vi "RT DAQ Settings.vi"(8 "error in (no error)":errorcluster, 9 "DAQ Trigger":T1={"Trig Source"=0, "Digital Trigger"=FALSE, "Trig Edge"=10171, "Pulse Line"=0, "Pulse On Time"=0} {"Pulse Line" items=["/Line0", "/Line1", "/Line2", "/Line3", "/Line4", "/Line5", "/Line6", "/Line7", "/Line8", "/Line9", "/Line10", "/Line11", "/Line12", "/Line13", "/Line14", "/Line15"]; "Trig Edge" items=["Rising"=10280, "Falling"=10171]; "Trig Source" items=["PFI0", "PFI1", "PFI2", "PFI3", "PFI4", "PFI5", "PFI6", "PFI7", "PFI8", "PFI9", "PFI10", "PFI11", "PFI12", "PFI13", "PFI14", "PFI15"]}, 10 "DAQ Timing":T2={"Number of Samples"=40000, "Samples Per Second"=970000.0, "Sample Mode"=10178, "Timeout (s)"=10.0} {"Sample Mode" items=["Continuous"=10123, "Finite Sample"=10178, "Hardware Timed Single Point"=12522]}, 11 "DAQ Channel":T3={"Channel"=1, "input terminal configuration"=10106, "Input Range Range"=10.0, "Device"="DAQ1"} {"input terminal configuration" items=["default"=-1, "RSE"=10083, "NRSE"=10078, "Differential"=10106, "Pseudodifferential"=12529]; "Input Range Range" items=["+/-10V"=10.0, "+/-5V"=5.0, "+/-2V"=2.0, "+/-1V"=1.0, "+/-0.5V"=0.5, "+/-0.2V"=0.2, "+/-0.1V"=0.1]; "Channel" items=["0"=0, "1"=1, "2"=2, "3"=3, "4"=4, "5"=5, "6"=6, "7"=7, "16"=16, "17"=17, "18"=18, "19"=19, "20"=20, "21"=21, "22"=22, "23"=23]}) -> (0 "error out":errorcluster, 1 "DAQ Trigger Out":T1={"Trig Source"=0, "Digital Trigger"=FALSE, "Trig Edge"=10171, "Pulse Line"=0, "Pulse On Time"=0} {"Pulse Line" items=["/Line0", "/Line1", "/Line2", "/Line3", "/Line4", "/Line5", "/Line6", "/Line7", "/Line8", "/Line9", "/Line10", "/Line11", "/Line12", "/Line13", "/Line14", "/Line15"]; "Trig Edge" items=["Rising"=10280, "Falling"=10171]; "Trig Source" items=["PFI0", "PFI1", "PFI2", "PFI3", "PFI4", "PFI5", "PFI6", "PFI7", "PFI8", "PFI9", "PFI10", "PFI11", "PFI12", "PFI13", "PFI14", "PFI15"]}, 2 "DAQ Timing Out":T2={"Number of Samples"=40000, "Samples Per Second"=970000.0, "Sample Mode"=10178, "Timeout (s)"=10.0} {"Sample Mode" items=["Continuous"=10123, "Finite Sample"=10178, "Hardware Timed Single Point"=12522]}, 3 "DAQ Channel  Out":T3={"Channel"=1, "input terminal configuration"=10106, "Input Range Range"=10.0, "Device"="DAQ1"} {"input terminal configuration" items=["default"=-1, "RSE"=10083, "NRSE"=10078, "Differential"=10106, "Pseudodifferential"=12529]; "Input Range Range" items=["+/-10V"=10.0, "+/-5V"=5.0, "+/-2V"=2.0, "+/-1V"=1.0, "+/-0.5V"=0.5, "+/-0.2V"=0.2, "+/-0.1V"=0.1]; "Channel" items=["0"=0, "1"=1, "2"=2, "3"=3, "4"=4, "5"=5, "6"=6, "7"=7, "16"=16, "17"=17, "18"=18, "19"=19, "20"=20, "21"=21, "22"=22, "23"=23]}, 7 "DAQ Pusle Out":T4)   [LabVIEW 2013]
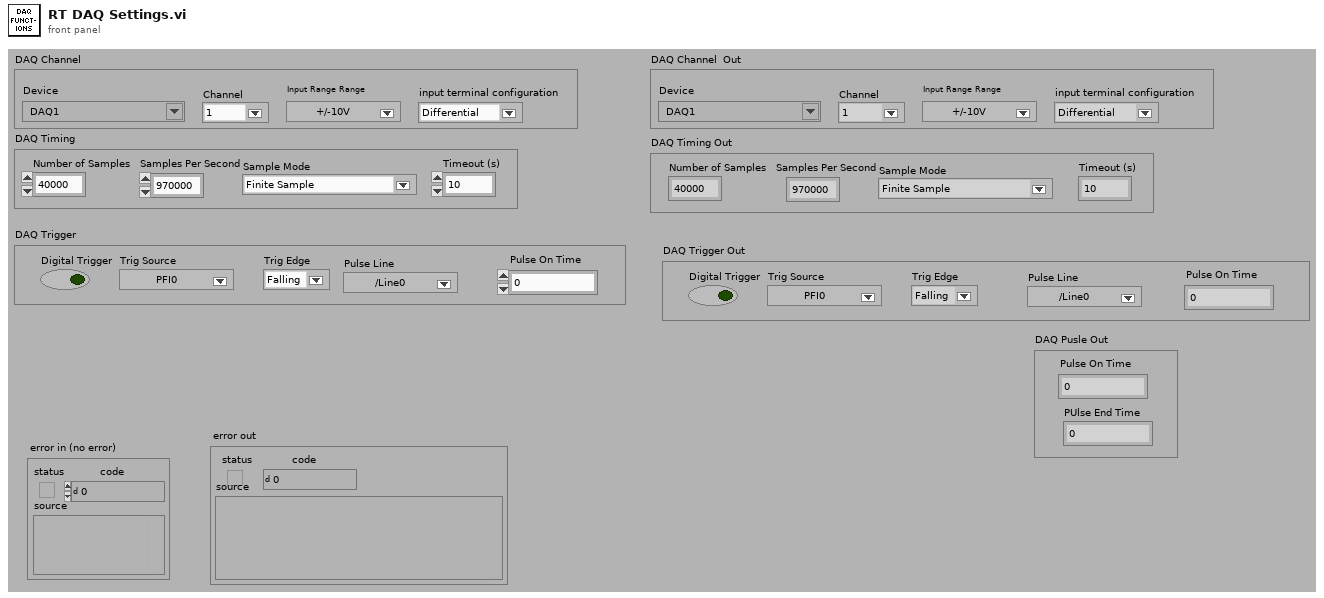
[diagram p1: front panel]
types:
  T1 = cluster{"Trig Source":u16, "Digital Trigger":bool, "Trig Edge":i32, "Pulse Line":u16, "Pulse On Time":u32}
  T2 = cluster{"Number of Samples":u32, "Samples Per Second":dbl, "Sample Mode":i32, "Timeout (s)":dbl}
  T3 = cluster{"Channel":u16, "input terminal configuration":i32, "Input Range Range":dbl, "Device":string}
  T4 = cluster{"Pulse On Time":u32, "PUlse End Time":u32}
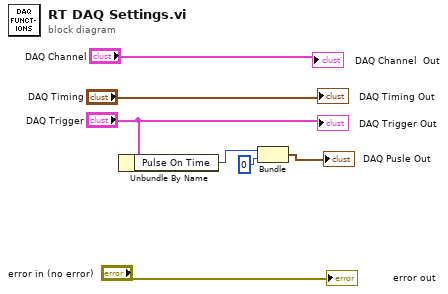
[diagram p0: block diagram]
diagram:
  n1 = Unbundle By Name("DAQ Trigger") -> ("Pulse On Time"=w2:u32)
  n2 = Bundle("Pulse On Time"=w2, 0) -> (→"DAQ Pusle Out":cluster{"Pulse On Time":u32, i32})  [unwired: 1 in]
  "error out" <- "error in (no error)"
  "DAQ Channel  Out" <- "DAQ Channel"
  "DAQ Timing Out" <- "DAQ Timing"
  "DAQ Trigger Out" <- "DAQ Trigger"
